vi "Bridge_Preempt.vi"(8 "error in (no error)":errorcluster={"status"=FALSE, "code"=0, "source"="\"\""}, 10 "active lease table":string, 11 "Fault latch":string) -> (0 "error out":errorcluster={"status"=FALSE, "code"=0, "source"="\"\""}, 2 "status ok":bool, 3 "Revocation events":string)   [LabVIEW 2026]
doc: "INTENT: Remove normal command authority on stop/fault. LOGIC: Invalidate tokens, flush/reject queued normal commands, request protective RT response."
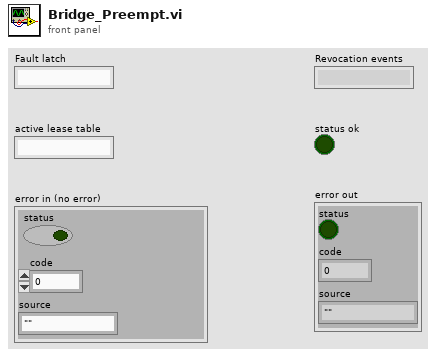
[diagram p1: front panel]
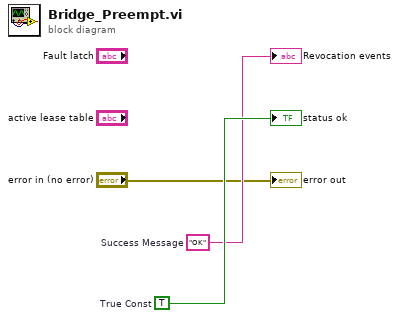
[diagram p0: block diagram]
diagram:
  w3 = TRUE  # True Const
  w2 = "OK"  # Success Message
  "Revocation events" <- w2
  "status ok" <- w3
  "error out" <- "error in (no error)"
